vi "News Ticker Text.vi"(10 "lines":i32=8, 11 "market":T1) -> (3 "text":string)   [LabVIEW 2020, in "Full Featured MCP Server.lvlib"]
doc: "Formats the latest news as text for the front panel: one line per item, newest on top, with its age in seconds."
uses:
  Full Featured MCP Server.lvlib
  Market State.ctl
  News Item.ctl
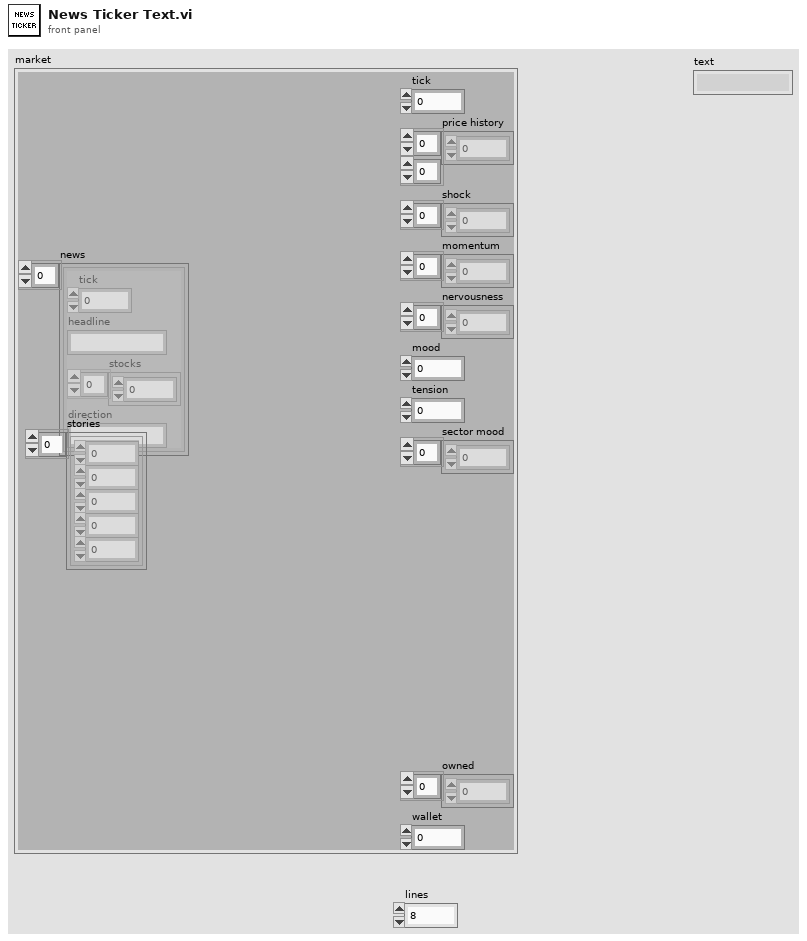
[diagram p1: front panel]
types:
  T1 = typedef "Full Featured MCP Server.lvlib/Market State.ctl" = cluster{"tick":i32, "price history":dbl[][], "shock":dbl[], "momentum":dbl[], "nervousness":dbl[], "mood":dbl, "tension":dbl, "sector mood":dbl[], "news":T2[], "stories":cluster{"arc":i32, "step":i32, "due":i32, "stock":i32, "other":i32}[], "owned":i32[], "wallet":dbl}
  T2 = typedef "Full Featured MCP Server.lvlib/News Item.ctl" = cluster{"tick":i32, "headline":string, "stocks":i32[], "direction":string}
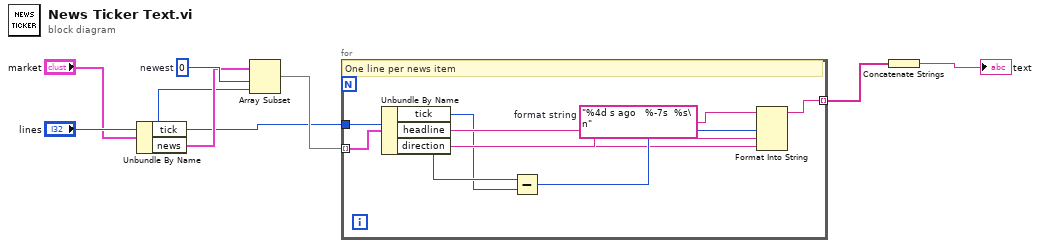
[diagram p0: block diagram]
diagram:
  w7 = 0  # newest
  n1 = Unbundle By Name("market") -> ("tick"=w3:i32, "news"=w4:T2[])
  n2 = Array Subset(array=w4, index=w7, length="lines") -> (w5:T2[])
  n3 = for {
    tunnel: w3 -> [w13]
    tunnel: w5 -> [w9] mode=indexing
    tunnel: [w16] -> w6 mode=indexing
    w15 = "%4d s ago   %-7s  %s\n"  # format string
    # "One line per news item"
    n4 = Unbundle By Name(w9) -> ("tick"=w10:i32, "headline"=w11:string, "direction"=w12:string)
    n5 = Subtract(x=w13, y=w10) -> (x-y=w14:i32)
    n6 = Format Into String(format string=w15, w14, w12, w11) -> (resulting string=w16:string)  [unwired: 2 in, 1 out]
  }
  n7 = Concatenate Strings(w6) -> (→"text":string)
